vi "Main.vi"() -> ()   [LabVIEW 2018, in "login.lvlib"]
doc: "This template is based from the Queued Message Handler design pattern and the Queued Message Handler Project Template that ships with LabVIEW 2014.\n\nThe main difference is that the Queue is private to this module and communication between modules is done via Broadcast and Request events.\n\nRequest events are wrapped via public API methods and are handled in the Event handler loop in this VI.\nAny module can register for Broadcast events sent by this module.\n\nThe Event Handling Loop generates messages based on user interface actions.\n\nThe Message Handling Loop processes messages generated by the Event Handling Loop, or by other messages. The messages are string values, so new messages can be added easily to the Message Cases case structure in the Message Handling Loop. Each message cluster can also provide an optional value for Message Data, which is a variant that can be converted to whatever message-specific data is required.\n_____\nBased on Delacor QMH Project Template 3.1.0.34."
uses:
  login.lvlib
  <vilib>/Delacor/Delacor QMH/Libraries/Module Admin_class/Delacor_lib_QMH_Module Admin.lvclass
  <vilib>/MGI/Panel Manager/Panel/Panel/Panel.lvclass
  <vilib>/Utility/miscctls.llb/LVPointTypeDef.ctl
  Module Data--cluster.ctl
  Database/Database_access.lvclass
  Path_Management_Class/Path_management.lvclass
  <vilib>/Delacor/Delacor QMH/Libraries/Message Queue_class/Delacor_lib_QMH_Message Queue.lvclass/Delacor_lib_QMH_Message Queue.ctl
  Stop Argument--cluster.ctl
  <vilib>/Delacor/Delacor QMH/Libraries/Module Admin_class/Delacor_lib_QMH_Module Admin.lvclass/Delacor_lib_QMH_Module Admin.ctl
  hid_panl Argument--cluster.ctl
  <vilib>/Utility/miscctls.llb/LVRowAndColumnTypeDef.ctl
  Path_Management_Class/Register_path.ctl
  <vilib>/Delacor/Delacor QMH/Libraries/Message Queue_class/Delacor_lib_QMH_Enqueue Message (Single).vi
  <vilib>/Delacor/Delacor QMH/Libraries/Module Admin_class/Delacor_lib_QMH_Get External Launch.vi
  <vilib>/MGI/Panel Manager/Panel/Panel/Window/Window.lvclass
  C:/Program Files (x86)/National Instruments/LabVIEW 2018/vi.lib/MGI/Panel Manager/Panel/Panel/Panel.lvclass
  <vilib>/Utility/error.llb/Error Cluster From Error Code.vi
  <vilib>/MGI/Panel Manager/Panel/Panel/Window/Window.vi
  <vilib>/ErrorRing/Error Ring.xnode
  <vilib>/Delacor/Delacor QMH/Libraries/Message Queue_class/Delacor_lib_QMH_Message Queue.lvclass
  <vilib>/MGI/Panel Manager/Panel/Panel Helper/Panel Helper.lvclass
  <vilib>/MGI/Panel Manager/Panel/Panel.lvlib
panel:
  in  "Panel 2":refnum<class "Panel.lvclass"> caption="Panel (Window)"
  in  "管理返回":bool
  in  "注册取消":bool
  in  "注册确定":bool
  in  "authority":u16(ring) items=["管理员", "操作员"]
  in  "Password":string
  in  "Name":string
  in  "用户信息":i32[](listbox)
  in  "注册":bool
  in  "删除":bool
  in  "改密确定":bool
  in  "改密取消":bool
  in  "确认新密码":string
  in  "新密码":string
  in  "旧密码":string
  out "用户名 2":string
  in  "返回":bool
  out "用户":string
  in  "退出登录":bool
  in  "用户管理":bool
  in  "修改密码":bool
  in  "登录取消":bool
  in  "登陆确定":bool
  in  "密码":string
  in  "用户名":string(combo)
  in  "Panel":refnum<class "Panel.lvclass">
  in  "Simulate MHL Error":bool
  in  "Simulate EHL Error":bool
  out "error out":errorcluster
  in  "Module Admin":refnum<class "Delacor_lib_QMH_Module Admin.lvclass">
  out "Status":string
  # "XXX登录系统"
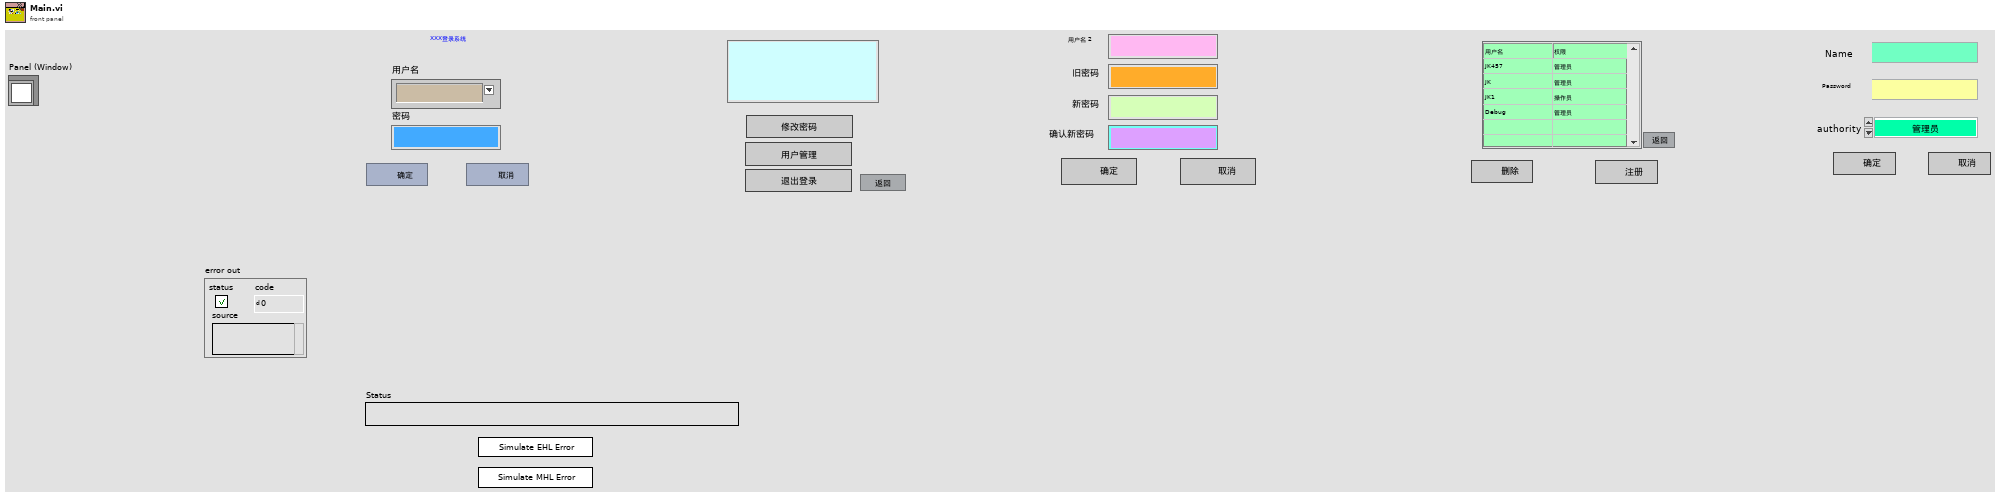
[diagram p1: front panel]
types:
  T1 = typedef "LVPointTypeDef.ctl" = cluster{"Horizontal":i16, "Vertical":i16}
  T2 = typedef "login.lvlib/Request Events--cluster.ctl" = cluster{"Stop Module":refnum<user-event>, "Show Panel":refnum<user-event>, "Hide Panel":refnum<user-event>, "Get Module Execution Status":refnum<user-event>, "Show Diagram":refnum<user-event>, "Change Panel":refnum<user-event>, "原点":refnum<user-event>, "hid_panl":refnum<user-event>}
  T3 = typedef "Panel.lvlib/Panel Helper.lvclass/Panel Events.ctl" = cluster{"My Panel":refnum<user-event>, "Top Level Initialized":refnum<user-event>}
  T4 = typedef "login.lvlib/Broadcast Events--cluster.ctl" = cluster{"Module Did Init":refnum<user-event>, "Status Updated":refnum<user-event>, "Error Reported":refnum<user-event>, "Module Did Stop":refnum<user-event>, "Update Module Execution Status":refnum<user-event>}
  T5 = typedef "login.lvlib/Module Data--cluster.ctl" = cluster{"Status":string, "Database_access.lvclass":refnum<class "Database_access.lvclass">, "Path_management.lvclass":refnum<class "Path_management.lvclass">, "user-passwords":string}
  T6 = typedef "login.lvlib/Stop Argument--cluster.ctl" = cluster{"Origin":string, "Exit via Stop Module Req?":bool, "Wait for Module to stop?":bool}
  T7 = typedef "login.lvlib/原点 Argument--cluster.ctl" = cluster{"x":dbl, "y":dbl}
  T8 = typedef "login.lvlib/hid_panl Argument--cluster.ctl" = cluster{"布尔":bool}
  T9 = typedef "LVRowAndColumnTypeDef.ctl" = cluster{"Row":i32, "Column":i32}
  T10 = typedef "Path_management.lvclass/Register_path.ctl" = string
  T11 = enum32{"invalid lock state", "Not Locked", "Locked (No Password)", "Password-protected"}
  T12 = enum32{"Invalid", "Standard", "Closed", "Hidden", "Minimized", "Maximized"}
  T13 = typedef "login.lvlib/登录蔟.ctl" = cluster{"登录名":string, "权限":string}
  T14 = cluster{"Name":string, "字符串":string, "Password":string}
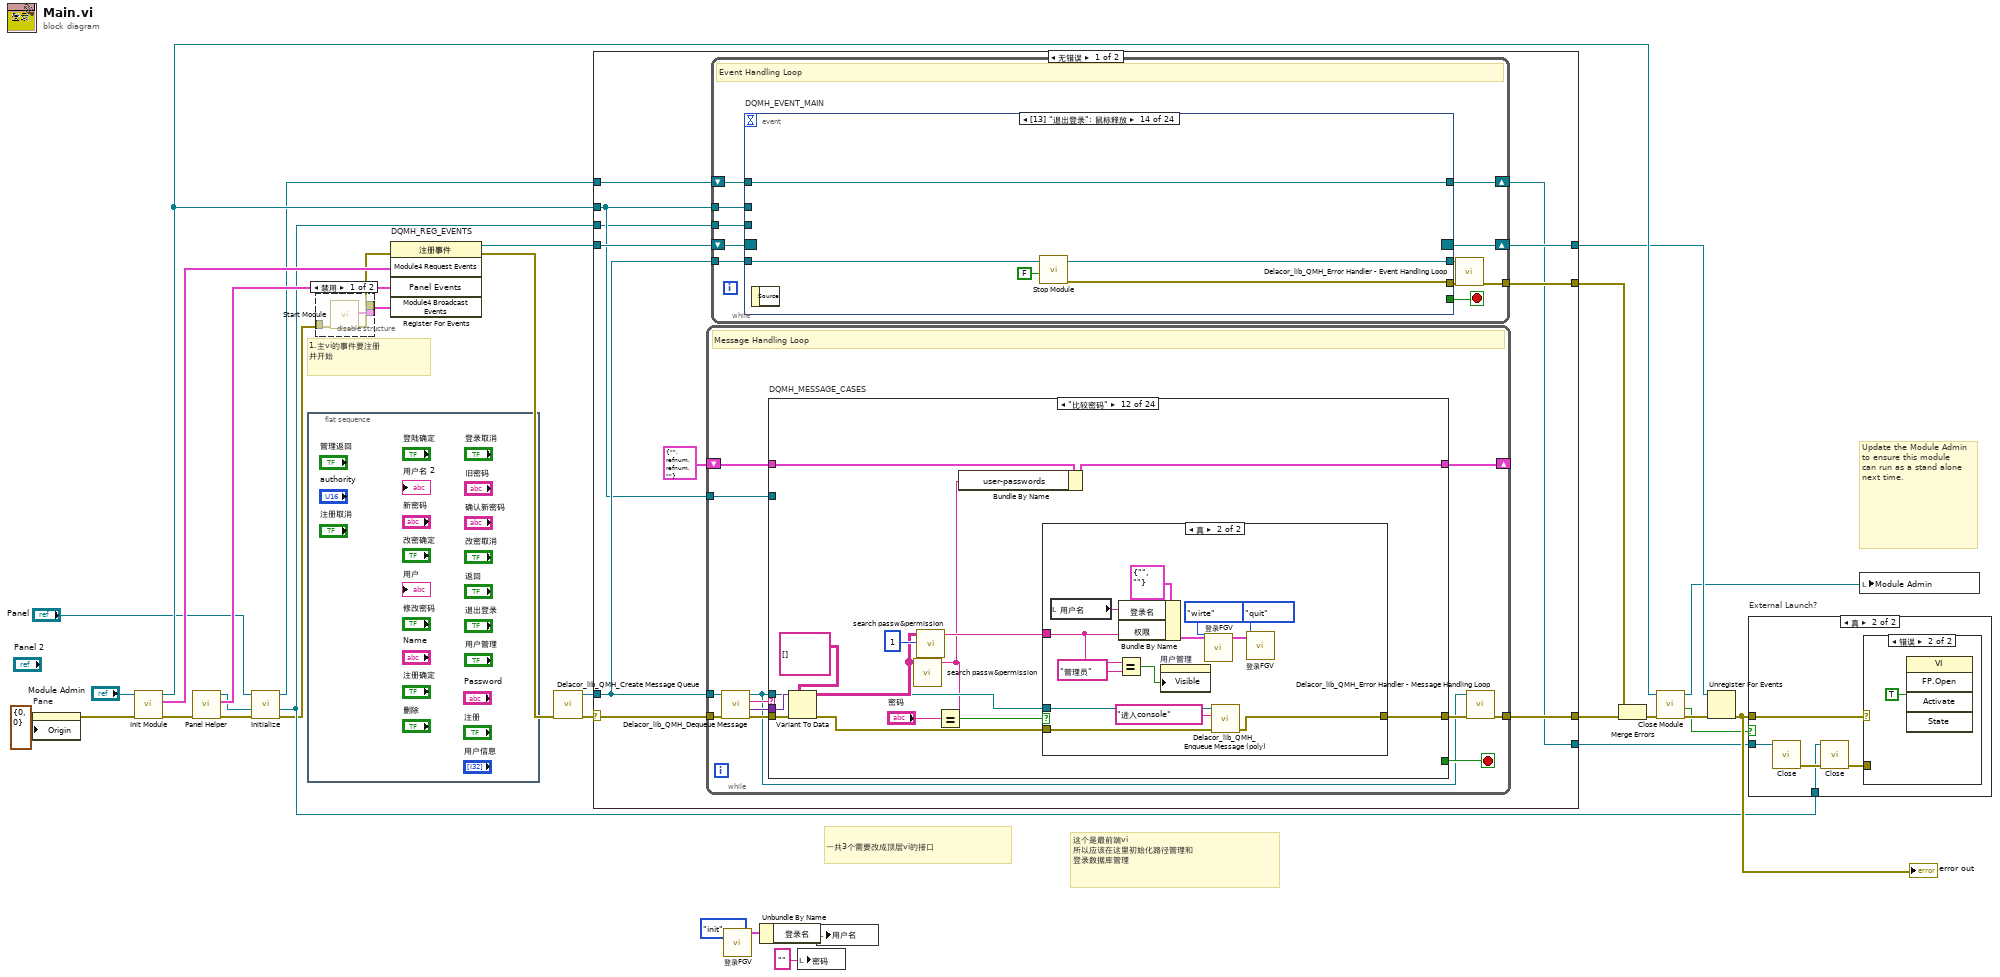
[diagram p0: block diagram]
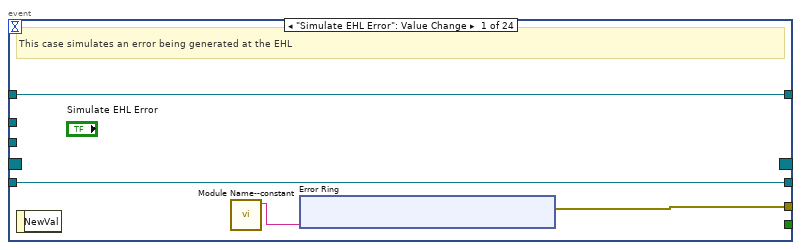
[diagram p5: hidden frame]
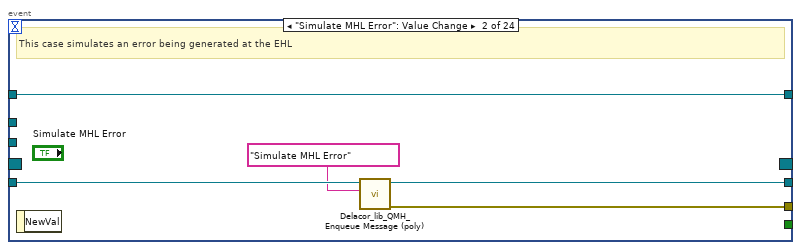
[diagram p6: hidden frame]
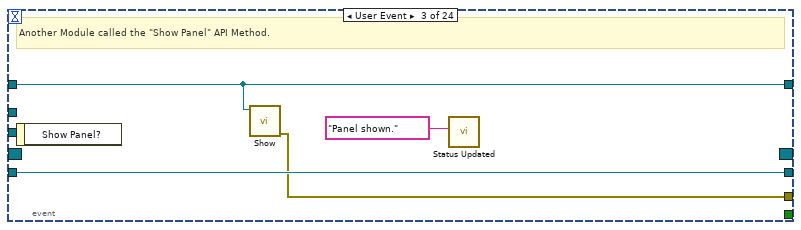
[diagram p7: hidden frame]
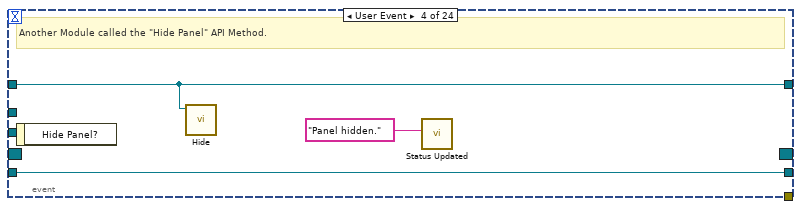
[diagram p8: hidden frame]
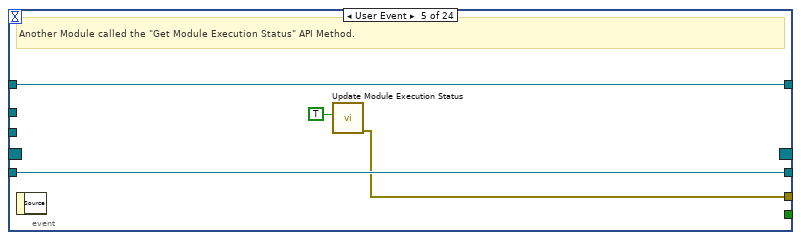
[diagram p9: hidden frame]
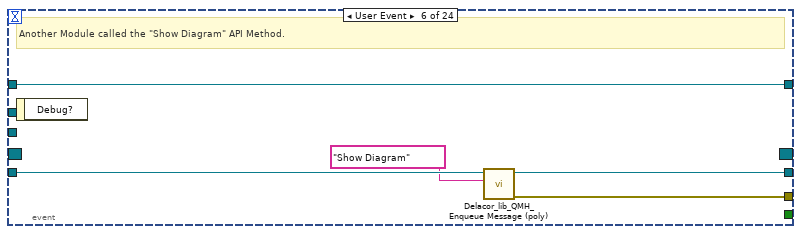
[diagram p10: hidden frame]
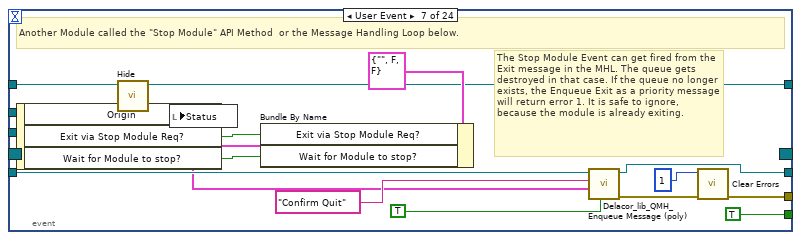
[diagram p11: hidden frame]
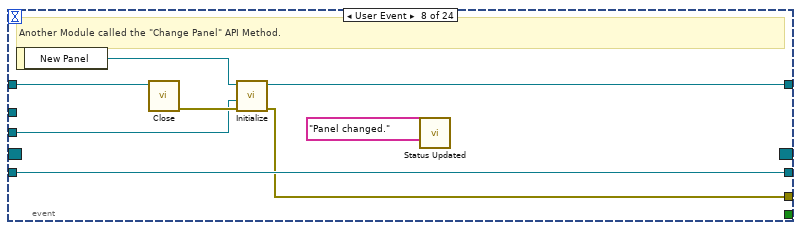
[diagram p12: hidden frame]
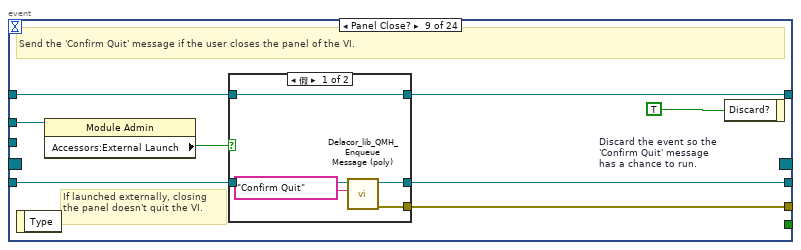
[diagram p13: hidden frame]
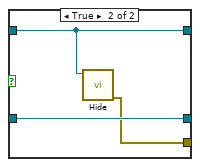
[diagram p14: hidden frame]
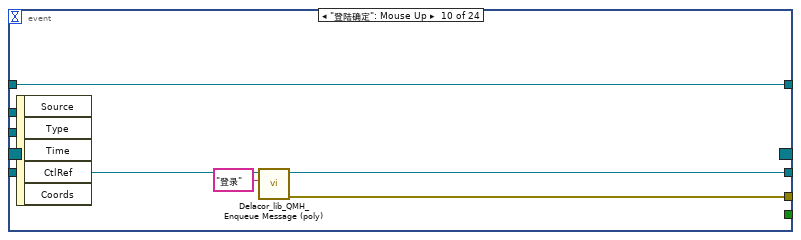
[diagram p15: hidden frame]
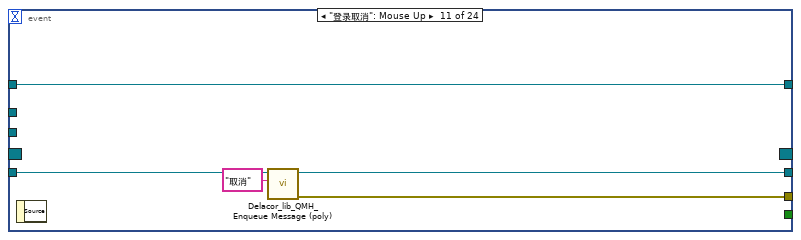
[diagram p16: hidden frame]
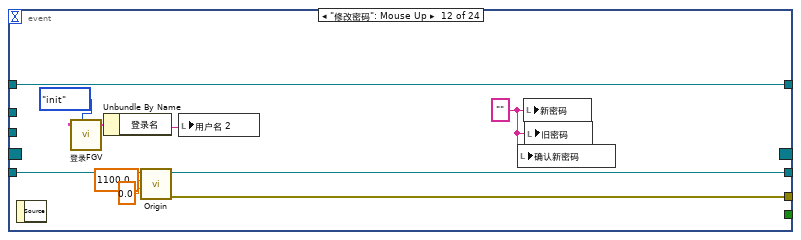
[diagram p17: hidden frame]
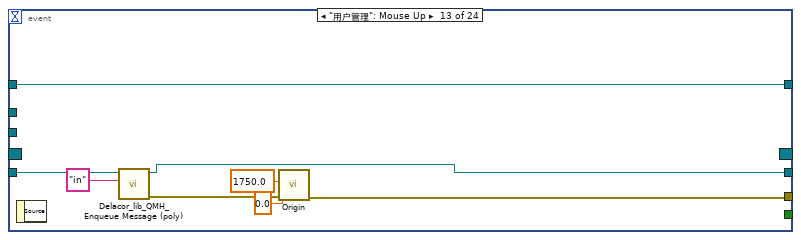
[diagram p18: hidden frame]
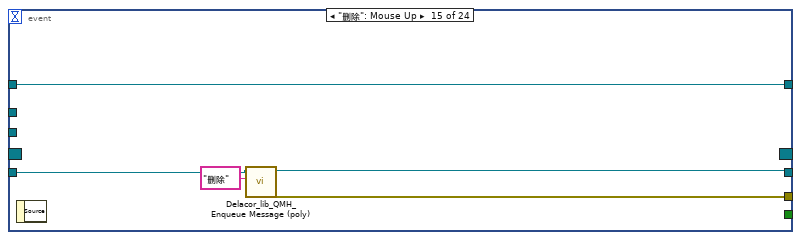
[diagram p19: hidden frame]
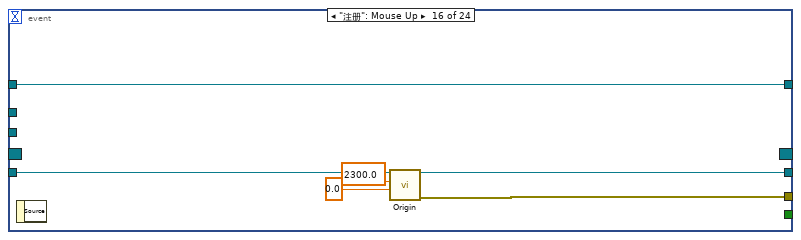
[diagram p20: hidden frame]
diagram:
  # "这个是最前端vi\n所以应该在这里初始化路径管理和\n登录数据库管理"
  # "一共3个需要改成顶层vi的接口"
  # "1.主vi的事件要注册\n并开始"
  # "Update the Module Admin to ensure this module can run as a stand alone next time."
  n1 = property on="Pane" class="Pane"("Origin"=T1 {"Horizontal"=0, "Vertical"=0}) -> (error out=w12:errorcluster)  [unwired: 2 in, 1 out]
  n2 = call "Init Module.vi"("error in (no error)"=w12, "Singleton Module Admin in"="Module Admin") -> ("error out"=w19:errorcluster, "Module4 Request Events"=w28:T2, "Singleton Module Admin out"=w32:refnum<class "Delacor_lib_QMH_Module Admin.lvclass">)  [unwired: 7 in]
  n3 = call <vilib>:"Panel Helper.vi"("Error In"=w19) -> ("Error Out"=w17:errorcluster, "Panel Events"=w18:T3, "Panel Helper out"=w16:refnum<class "Panel Helper.lvclass">)  [unwired: 8 in]
  n4 = call <vilib>:"Initialize.vi"("error in (no error)"=w17, "My Helper in"=w16, "Panel In"="Panel") -> ("error out"=w6:errorcluster, "My Helper out"=w15:refnum<class "Panel Helper.lvclass">, "Panel Out"=w14:refnum<class "Panel.lvclass">)  [unwired: 6 in]
  n5 = flat-sequence {
    frame #0 {
    }
  }
  n6 = disable-structure shown="禁用" {
    disable-tunnel: [w35 _] -> w8
    disable-tunnel: [w34 _] -> w7
    disable-tunnel: w6 -> [w33 _]
    frame Disabled {
      n7 = call "Start Module.vi"("error in (no error)"=w33) -> ("error out"=w34:errorcluster, "Module4 Broadcast Events"=w35:T4)  [unwired: 7 in, 2 out]
    }
    frame Enabled {
    }
  }
  n8 = register-events "DQMH_REG_EVENTS"(error in=w7, w28, w18, w8) -> (reference out=w29:refnum<event-registration>, error out=w5:errorcluster)  [unwired: 1 in]
  n9 = call <vilib>:"Delacor_lib_QMH_Create Message Queue.vi"("error in"=w5) -> ("error out"=w21:errorcluster, "Message Queue"=w27:refnum<class "Delacor_lib_QMH_Message Queue.lvclass">)  [unwired: 9 in]
  n10 = case shown="无错误" w21 {
    selector: w21 -> [w40 w566]
    tunnel: [w46 w566] -> w31
    tunnel: [w45 w571] -> w30
    tunnel: w29 -> [w43 w571]
    tunnel: w27 -> [w42 _]
    tunnel: [w41 _] -> w10
    tunnel: w32 -> [w39 w567]
    tunnel: w14 -> [w37 w563]
    tunnel: w15 -> [w38 _]
    tunnel: [w36 w563] -> w20
    frame No Error {
      n11 = while {
        tunnel: w42 -> [w219]
        shift-right: [w225] -> _
        shift-left: T5 {"Status"="", "Database_access.lvclass"=refnum, "Path_management.lvclass"=refnum, "user-passwords"=""} ("Data Cluster") -> [w226]
        tunnel: w40 -> [w223]
        tunnel: [w217] -> w46
        tunnel: w39 -> [w216]
        stop <- w224 stop-if-true
        # "Message Handling Loop"
        n12 = call-dynamic "Delacor_lib_QMH_Dequeue Message.vi"("error in"=w223, "Message Queue in"=w219) -> ("error out"=w222:errorcluster, "Message Data"=w220:variant, "Message"=w221:string, "Message Queue out"=w218:refnum<class "Delacor_lib_QMH_Message Queue.lvclass">)  [unwired: 6 in]
        n13 = case "DQMH_MESSAGE_CASES" shown="\"比较密码\"" w221 {
          selector: w221 -> [_ _ _ _ _ _ _ _ _ _ _ _ _ _ _ _ _ _ _ _ _ _ _ w552]
          tunnel: w218 -> [w229 w242 w262 _ _ _ _ _ _ _ w351 w373 _ _ w414 _ w463 w471 _ _ w516 w532 w548 _]
          tunnel: w222 -> [w231 w244 w261 w287 w299 w303 w321 w336 w344 w347 w349 w383 w402 w409 w415 w441 w464 w470 w500 w505 w522 w536 w550 _]
          tunnel: [w235 w249 w259 w280 w300 w302 w319 w334 w342 w345 w348 w374 w400 w406 w413 w439 w455 w475 w498 w503 w513 w534 w544 w553] -> w227
          tunnel: w226 -> [w240 w247 w265 w289 w301 w304 w320 w335 w343 w346 w350 w384 w403 w410 w417 w450 w461 w473 w499 w504 w521 w535 w547 w554]
          tunnel: [w239 w246 w264 w289 w301 w304 w320 w335 w343 w346 w350 w372 w403 w410 w417 w450 w461 w473 w499 w504 w521 w535 w547 w554] -> w225
          tunnel: [_ _ _ _ _ _ _ _ _ _ _ _ _ _ _ _ _ _ _ _ _ _ w546 _] -> w224
          tunnel: w220 -> [_ _ _ _ w298 _ _ w333 w341 _ _ w382 _ _ _ _ _ _ _ _ w520 _ w543 _]
          tunnel: w216 -> [w233 _ _ _ _ _ _ _ _ _ _ _ _ _ _ _ _ _ _ _ w515 _ w538 _]
          frame "Initialize" {
            w238 = "Initial Message" ("Initial Message")
            # "#CodeNeeded - Initialize the appearance of the front panel."
            # "#CodeNeeded - Initialize your state data here."
            # "Initialize - Any operation that needs to be done before the module can receive messages. Synchronize Caller Events.vi will inform Start Module.vi that the module has launched and is ready to receive messages. Module Did Init.vi will broadcast that the module initialized."
            n14 = call-poly <vilib>:"Delacor_lib_QMH_Enqueue Message (poly).vi"("error in"=w231, "Message"="init", "Message Queue in"=w229) -> ("error out"=w230:errorcluster)  [unwired: 7 in, 1 out]
            n15 = call "Show Panel.vi"("error in (no error)"=w230) -> ("error out"=w232:errorcluster)  [unwired: 10 in]
            n16 = call "Synchronize Caller Events.vi"("error in (no error)"=w232, "Singleton Module Admin in"=w233) -> ("error out"=w234:errorcluster)  [unwired: 8 in, 1 out]
            n17 = Bundle By Name(cluster=w240, "Status"=w238) -> (w239:T5)
            n18 = local write "Status"(w238) -> ()
            n19 = call "Module Name--constant.vi"() -> ("Module Name"=w236:string)  [unwired: 11 in]
            n20 = call "Module Did Init.vi"("error in (no error)"=w234, "Initialized?"=TRUE, "Origin"=w236) -> ("error out"=w235:errorcluster)  [unwired: 8 in]
          }
          frame "init" {
            n21 = call-poly <vilib>:"Delacor_lib_QMH_Enqueue Message (poly).vi"("error in"=w244, "Message"="ini", "Message Queue in"=w242) -> ("error out"=w243:errorcluster)  [unwired: 7 in, 1 out]
            n22 = in-place {
              in-place-border: w243 -> [w254]
              in-place-border: [w253] -> w245
              # "初始化路径管理类"
              n23 = in-place-cluster #1(w247) -> ("Path_management.lvclass"=w256:refnum<class "Path_management.lvclass">)
              n24 = call-dynamic "INIT_path.vi"("error in (no error)"=w254, "Path_management 输入"=w256) -> ("error out"=w253:errorcluster, "Path_management 输出"=w255:refnum<class "Path_management.lvclass">)  [unwired: 8 in]
              n25 = in-place-cluster #1("Path_management.lvclass"=w255) -> (w246:T5)
            }
            n26 = call-poly <vilib>:"Panel Type Selector.vi"("Default Title"="Window Test") -> ("error out"=w250:errorcluster, "Window out"=w251:refnum<class "Window.lvclass">)  [unwired: 9 in]
            n27 = call "Change Panel.vi"("error in (no error)"=w250, "New Panel"=w251) -> ("error out"=w248:errorcluster)  [unwired: 9 in]
            n28 = Merge Errors(w245, w248, w243) -> (w249:errorcluster)
          }
          frame "ini" {
            n29 = call-poly <vilib>:"Delacor_lib_QMH_Enqueue Message (poly).vi"("error in"=w261, "Message"="in", "Message Queue in"=w262) -> ("error out"=w260:errorcluster)  [unwired: 7 in, 1 out]
            n30 = in-place {
              in-place-border: w260 -> [w275]
              in-place-border: [w274] -> w259
              # "读出所有账户名"
              n31 = in-place-cluster #2(w265) -> ("Database_access.lvclass"=w278:refnum<class "Database_access.lvclass">)
              n32 = call "Take_Path.vi"("组合框"=T10 "登录数据库路径") -> ("Your_Path"=w277:path)  [unwired: 10 in]
              n33 = call-dynamic "INIT-Connect.vi"("error in (no error)"=w275, "database-path"=w277, "Database_access 输入"=w278) -> ("error out"=w274:errorcluster, "Database_access 输出"=w276:refnum<class "Database_access.lvclass">)  [unwired: 7 in]
              n34 = in-place-cluster #2("Database_access.lvclass"=w276) -> (w264:T5)
            }
            n35 = for {
              tunnel: T9 {"Row"=0, "Column"=0} ("活动单元格:活动单元格") -> [w268]
              tunnel: i32[] [0, 1] -> [w267] mode=indexing
              n36 = for {
                N: 99 -> [_]
                tunnel: w268 -> [w271]
                tunnel: w267 -> [w269]
                i -> [w270]
                n37 = Bundle By Name(cluster=w271, "Column"=w269, "Row"=w270) -> (w272:T9)
                n38 = property on="用户信息" class="MCListbox (严格)"("ActiveCell"=w272, "Justify"=enum16{"Left", "Center", "Right"}."Center" ("活动单元格:单元格对齐")) -> ()  [unwired: 2 in, 2 out]
              }
            }
          }
          frame "in" {
            n39 = Unbundle By Name(w289) -> ("Database_access.lvclass"=w288:refnum<class "Database_access.lvclass">)
            n40 = call-dynamic "Read_database.vi"("error in (no error)"=w287, "columns"=string[] ["User_Name", "User_Right"] ("table"), "table"="User_Table", "Database_access 输入"=w288) -> ("error out"=w285:errorcluster, "data"=w286:variant[][])  [unwired: 5 in, 1 out]
            n41 = call "StringArr-type"("error in (no error)"=w285, "database variant"=w286) -> ("error out"=w284:errorcluster, "data"=w283:string[][])  [unwired: 8 in]
            n42 = Index Array(array=w283, index (col)=0 ("禁用的索引 (列)")) -> (element=w293:string[])  [unwired: 1 in]
            n43 = property on="用户信息" class="MCListbox (严格)"("ItemNames"=w283) -> (error out=w281:errorcluster)  [unwired: 2 in, 1 out]
            n44 = property on="用户名" class="CmbBox"(error in=w284, "Strings[]"=w293) -> (error out=w282:errorcluster)  [unwired: 1 in, 1 out]
            n45 = Merge Errors(w282, w281) -> (w280:errorcluster)
          }
          frame "Update Display" {
            # "Broadcast updated status to any VI registered to listen to this module's broadcast events."
            # "Convert the message data to a string to display in the Status indicator."
            # "#CodeRecommended - If you wish to decouple the Message Handling Loop from your user interface, consider creating User Events (like the \"Stop\" event in this VI) to message the Event Handling Loop whenever the user interface needs updating."
            # "Update Display - Update user interface here."
            n46 = Variant To Data(error in=w299, type="" ("空字符串常量"), Variant=w298) -> (data=w296:string, error out=w295:errorcluster)
            "Status" <- w296
            n47 = call "Status Updated.vi"("error in (no error)"=w295, "Status"=w296) -> ("error out"=w294:errorcluster)  [unwired: 9 in]
            n48 = Merge Errors(w294) -> (w300:errorcluster)
          }
          frame "Show Diagram" {
            # "Show Diagram - Show the block diagram of this VI. Used as a debugging tool. There is a button in the module tester that fires the Show Diagram request, which runs this message. Note that the diagram will not be displayed if it is password-protected and the password is not in the cache."
            n49 = disable-structure shown="RUN_TIME_ENGINE==False" {
              disable-tunnel: [w312 w318] -> w302
              disable-tunnel: w303 -> [w311 w318]
              frame condition #0 (active) {
                # "functionality not available in exe"
                n50 = invoke class="VI" method="Lock State.Get"(error in=w311) -> (error out=w310:errorcluster, "Get Lock State"=w309:T11, "pwd in cache"=w306:bool)  [unwired: 3 in, 1 out]
                n51 = Equal?(x=T11."Password-protected", y=w309) -> (x = y?=w307:bool)
                n52 = Compound Arithmetic op=AND(w307, invert w306) -> (w305:bool)
                n53 = case shown="假" w305 {
                  tunnel: [w315 w317] -> w312
                  tunnel: w310 -> [w313 w317]
                  frame False {
                    n54 = property class="VI"(error in=w313, "BDWin.Open"=TRUE ("Block Diagram Window:Open")) -> (error out=w315:errorcluster)  [unwired: 1 in, 1 out]
                    n55 = call "Status Updated.vi"("Status"="Block Diagram shown." ("format string")) -> ()  [unwired: 10 in, 1 out]
                  }
                  frame True {
                    # "Password-protected VI, and the password is not in the cache. Do not show the diagram."
                  }
                }
              }
              frame condition #1 {
              }
            }
          }
          frame "--- Module Specific ---" {
            # "Separator -- The following cases handle messages specific to this Module."
            n56 = Merge Errors(w321) -> (w319:errorcluster)
          }
          frame "原点" {
            # "原点滚动"
            n57 = Variant To Data(error in=w336, type=T7 {"x"=0.0, "y"=0.0} ("原点 Argument"), Variant=w333) -> (data=w331:T7, error out=w334:errorcluster)
            n58 = Unbundle By Name(w331) -> ("x"=w328:dbl, "y"=w327:dbl)
            n59 = Bundle By Name(cluster=T1 {"Horizontal"=0, "Vertical"=0} ("原点"), "Horizontal"=w328, "Vertical"=w327) -> (w329:T1)
            n60 = call "登录FGV.vi"("枚举"=enum16{"init", "quit", "read", "wirte"}."read") -> ("wirte 2"=w325:T13)  [unwired: 10 in]
            n61 = Unbundle By Name(w325) -> ("登录名"=w324:string)
            n62 = property on="Pane" class="Pane"("Origin"=w329) -> ()  [unwired: 2 in, 2 out]
            n63 = Format Into String(format string="欢迎--QAQ--\n%s\n花花Cillao花花" ("格式字符串"), w324) -> (resulting string=w323:string)  [unwired: 2 in, 1 out]
            n64 = local write "用户"(w323) -> ()
          }
          frame "hid_panl" {
            # "内部调用前面板关闭会出问题，我就自己写了一个简单的\n这个只内部调用"
            n65 = Variant To Data(error in=w344, type=T8 {"布尔"=FALSE} ("hid_panl Argument"), Variant=w341) -> (data=w339:T8, error out=w342:errorcluster)
            n66 = Unbundle By Name(w339) -> ()  [unwired: 1 out]
            n67 = control-ref of="本VI"() -> (w338:refnum<vi>)
            n68 = invoke class="VI" method="FP.Open"(reference=w338, "State"=T12."Hidden" ("状态")) -> ()  [unwired: 3 in, 5 out]
          }
          frame "---Copy This Frame---" {
            # "Duplicate this frame when creating new messages.  Change this comment in the duplicated frame to describe this message."
            n69 = Merge Errors(w347) -> (w345:errorcluster)
          }
          frame "登录" {
            n70 = Empty String/Path?(string/path="用户名") -> (empty?=w353:bool)
            n71 = case shown="假" w353 {
              tunnel: "用户名" -> [w362 _]
              tunnel: w351 -> [w368 _]
              tunnel: w350 -> [w367 _]
              tunnel: w349 -> [w360 w369]
              tunnel: [w358 w369] -> w348
              frame False {
                n72 = Unbundle By Name(w367) -> ("Database_access.lvclass"=w366:refnum<class "Database_access.lvclass">)
                n73 = Format Into String(format string=" where User_Name ='%s'" ("condition"), error in=w360, w362) -> (resulting string=w361:string, error out=w359:errorcluster)  [unwired: 1 in]
                n74 = call-dynamic "Read_database.vi"("condition"=w361, "error in (no error)"=w359, "table"="User_Table", "Database_access 输入"=w366) -> ("error out"=w356:errorcluster, "data"=w357:variant[][])  [unwired: 5 in, 1 out]
                n75 = call "StringArr-type"("error in (no error)"=w356, "database variant"=w357) -> ("error out"=w355:errorcluster, "data"=w354:string[][])  [unwired: 8 in]
                n76 = call-poly <vilib>:"Delacor_lib_QMH_Enqueue Message (poly).vi"("error in"=w355, "Message Data"=w354, "Message"="比较密码", "Message Queue in"=w368) -> ("error out"=w358:errorcluster)  [unwired: 6 in, 1 out]
              }
              frame True {
                n77 = One Button Dialog(message="我都弄成让你选的了\n你还不输入的话很难办啊盆友" ("消息")) -> ()  [unwired: 1 in, 1 out]
              }
            }
          }
          frame "比较密码" {
            n78 = Variant To Data(error in=w383, type=string[][] [] ("table"), Variant=w382) -> (data=w378:string[][], error out=w375:errorcluster)
            n79 = call "search passw&permission.vi"("数组"=w378) -> ("元素"=w371:string)  [unwired: 9 in, 1 out]
            n80 = call "search passw&permission.vi"("索引"=1, "数组"=w378) -> ("元素"=w376:string)  [unwired: 8 in, 1 out]
            n81 = Equal?(x=w371, y="密码") -> (x = y?=w377:bool)
            n82 = Bundle By Name(cluster=w384, "user-passwords"=w371) -> (w372:T5)
            n83 = case shown="真" w377 {
              tunnel: w376 -> [_ w389]
              tunnel: w375 -> [w386 w393]
              tunnel: [w386 w392] -> w374
              tunnel: w373 -> [_ w391]
              frame False {
                n84 = One Button Dialog(message="是本人吗就乱登录" ("消息")) -> ()  [unwired: 1 in, 1 out]
              }
              frame True {
                n85 = local read "用户名"() -> (w394:string)
                n86 = Equal?(x=w389, y="管理员") -> (x = y?=w388:bool)
                n87 = Bundle By Name(cluster=T13 {"登录名"="", "权限"=""} ("wirte"), "登录名"=w394, "权限"=w389) -> (w398:T13)
                n88 = property on="用户管理" class="Bool (严格)"("Visible"=w388) -> ()  [unwired: 2 in, 2 out]
                n89 = call "登录FGV.vi"("枚举"=enum16{"init", "quit", "read", "wirte"}."wirte", "wirte"=w398) -> ("wirte 2"=w399:T13)  [unwired: 9 in]
                n90 = call-poly <vilib>:"Delacor_lib_QMH_Enqueue Message (poly).vi"("error in"=w393, "Message"="进入console", "Message Queue in"=w391) -> ("error out"=w392:errorcluster)  [unwired: 7 in, 1 out]
                n91 = call "登录FGV.vi"("枚举"=enum16{"init", "quit", "read", "wirte"}."quit", "wirte"=w399) -> ()  [unwired: 9 in, 1 out]
              }
            }
          }
          frame "进入console" {
            # "2.进入时候打开主vi面板"
            # "隐藏自己"
            # "展示main"
            n92 = call "Hide Panel.vi"("error in (no error)"=w402) -> ("error out"=w401:errorcluster)  [unwired: 10 in]
            n93 = disable-structure shown="禁用" {
              disable-tunnel: w401 -> [w405 _]
              disable-tunnel: [w404 _] -> w400
              frame Disabled {
                n94 = call "Show Panel.vi"("error in (no error)"=w405) -> ("error out"=w404:errorcluster)  [unwired: 10 in]
              }
              frame Enabled {
              }
            }
          }
          frame "取消" {
            # "3.停止主VI"
            # "停止"
            # "隐藏自己"
            # "为什么要先隐藏\n因为再DQMH中只有点X号才能\n出发关闭前面板，否则会变成停止，"
            n95 = call "Hide Panel.vi"("error in (no error)"=w409) -> ("error out"=w408:errorcluster)  [unwired: 10 in]
            n96 = disable-structure shown="禁用" {
              disable-tunnel: w408 -> [w412 _]
              disable-tunnel: [w411 _] -> w407
              frame Disabled {
                n97 = call "Stop Module.vi"("error in (no error)"=w412) -> ("error out"=w411:errorcluster)  [unwired: 10 in]
              }
              frame Enabled {
              }
            }
            n98 = call "Stop Module.vi"("error in (no error)"=w407) -> ("error out"=w406:errorcluster)  [unwired: 10 in]
          }
          frame "修改密码" {
            w423 = "" ("y")
            n99 = local read "确认新密码"() -> (w424:string)
            n100 = Unbundle By Name(w417) -> ("user-passwords"=w416:string)
            n101 = local read "新密码"() -> (w418:string)
            n102 = Equal?(x=w418, y=w424) -> (x = y?=w422:bool)
            n103 = Not Equal?(x=w418, y=w423) -> (x != y?=w421:bool)
            n104 = Not Equal?(x=w423, y=w424) -> (x != y?=w420:bool)
            n105 = local read "旧密码"() -> (w426:string)
            n106 = Compound Arithmetic op=AND ("复合运算")(w422, w421, w420) -> (w419:bool)
            n107 = Equal?(x=w416, y=w426) -> (x = y?=w425:bool)
            n108 = case shown="真" w425 {
              tunnel: w419 -> [_ w432]
              tunnel: w418 -> [_ _]
              tunnel: w415 -> [w427 w430]
              tunnel: w414 -> [_ w431]
              tunnel: [w427 w429] -> w413
              frame False {
                n109 = One Button Dialog(message="要输入正确原始密码\n才可以呦" ("消息")) -> ()  [unwired: 1 in, 1 out]
              }
              frame True {
                n110 = case shown="真" w432 {
                  tunnel: w431 -> [_ w438]
                  tunnel: w430 -> [w433 w437]
                  tunnel: [w433 w435] -> w429
                  frame False {
                    n111 = One Button Dialog(message="两次输的\n不一样啊" ("消息")) -> ()  [unwired: 1 in, 1 out]
                  }
                  frame True {
                    n112 = call-poly <vilib>:"Delacor_lib_QMH_Enqueue Message (poly).vi"("error in"=w437, "Message"="修改数据库", "Message Queue in"=w438) -> ("error out"=w435:errorcluster)  [unwired: 7 in, 1 out]
                  }
                }
              }
            }
          }
          frame "修改数据库" {
            n113 = Unbundle By Name(w450) -> ("Database_access.lvclass"=w449:refnum<class "Database_access.lvclass">)
            n114 = local read "用户名 2"() -> (w444:string)
            n115 = Format Into String(format string="Where User_Name='%S'", error in=w441, w444) -> (resulting string=w443:string, error out=w442:errorcluster)  [unwired: 1 in]
            n116 = local read "新密码"() -> (w446:string)
            n117 = call-dynamic "Update_database.vi"("data"=w446, "condition"=w443, "error in (no error)"=w442, "columns"=string[] ["User_Password"], "table"="User_Table", "Database_access 输入"=w449) -> ("error out"=w440:errorcluster)  [unwired: 4 in, 1 out]
            n118 = call "Origin.vi"("error in"=w440, "数值 2"=0.0, "数值"=550.0) -> ("error out"=w439:errorcluster)  [unwired: 8 in]
            n119 = One Button Dialog(message="密码已修改" ("消息"), button name ("OK")="朕知道了" ("按钮名称（“确定”）")) -> ()  [unwired: 1 out]
          }
          frame "删除" {
            n120 = Unbundle By Name(w461) -> ("Database_access.lvclass"=w460:refnum<class "Database_access.lvclass">)
            n121 = call-poly <vilib>:"Delacor_lib_QMH_Enqueue Message (poly).vi"("error in"=w464, "Message"="in", "Message Queue in"=w463) -> ("error out"=w458:errorcluster)  [unwired: 7 in, 1 out]
            n122 = property on="用户信息" class="MCListbox (严格)"() -> ("ItemNames"=w466:string[][], "FocusRow"=w467:i32)  [unwired: 2 in, 2 out]
            n123 = Index Array(array=w466, index (row)=w467) -> (element=w465:string[])  [unwired: 1 in]
            n124 = Index Array(array=w465) -> (element=w456:string)  [unwired: 1 in]
            n125 = call-dynamic "Delete_database.vi"("name"=w456, "error in (no error)"=w458, "Item-name"="User_Name" ("table"), "table"="User_Table", "Database_access 输入"=w460) -> ("error out"=w455:errorcluster)  [unwired: 5 in, 1 out]
          }
          frame "注册确定" {
            n126 = local read "Password"() -> (w468:string)
            n127 = local read "Name"() -> (w474:string)
            n128 = local read "authority"() -> (w477:u16)
            n129 = Empty String/Path?(string/path=w474) -> (empty?=w479:bool)
            n130 = Empty String/Path?(string/path=w468) -> (empty?=w480:bool)
            n131 = call "emur-char.vi"("authority 2"=w477) -> ("字符串"=w476:string)  [unwired: 10 in]
            n132 = Not And(1:w480, 2:w479) -> (0:w478:bool)
            n133 = case shown="真" w478 {
              tunnel: w476 -> [_ w482]
              tunnel: w474 -> [_ w496]
              tunnel: w468 -> [_ w483]
              tunnel: w473 -> [_ w497]
              tunnel: [_ w488] -> w472
              tunnel: w471 -> [_ w487]
              tunnel: w470 -> [_ w495]
              tunnel: [_ w485] -> w469
              frame False {
                n134 = One Button Dialog(message="不能有空的啊" ("消息")) -> ()  [unwired: 1 in, 1 out]
              }
              frame True {
                n135 = Unbundle By Name(w497) -> ("Database_access.lvclass"=w492:refnum<class "Database_access.lvclass">)
                n136 = Bundle("Name"=w496, "字符串"=w482, "Password"=w483) -> (w489:T14)  [unwired: 1 in]
                n137 = call "Origin.vi"("error in"=w495, "数值 2"=0.0, "数值"=1750.0) -> ("error out"=w486:errorcluster)  [unwired: 8 in]
                n138 = call-dynamic "Insert_database.vi"("data"=w489, "columns"=string[] ["User_name", "User_Right", "User_password"], "table"="User_Table", "Database_access 输入"=w492) -> ("error out"=w488:errorcluster)  [unwired: 6 in, 1 out]
                n139 = call-poly <vilib>:"Delacor_lib_QMH_Enqueue Message (poly).vi"("error in"=w486, "Message"="in", "Message Queue in"=w487) -> ("error out"=w485:errorcluster)  [unwired: 7 in, 1 out]
              }
            }
            n140 = Merge Errors(w472, w469) -> (w475:errorcluster)
          }
          frame "--- Exit and Error Handling---" {
            # "Separator - The following cases handle errors and exit messages."
            n141 = Merge Errors(w500) -> (w498:errorcluster)
          }
          frame "Simulate MHL Error" {
            # "Simulate an error occurring at the MHL"
            n142 = call "Module Name--constant.vi"() -> ("Module Name"=w502:string)  [unwired: 11 in]
            n143 = xnode "Error Ring"("参数 0"=w502) -> ("错误输出"=w501:errorcluster)
            n144 = Merge Errors(w505, w501) -> (w503:errorcluster)
          }
          frame "Error" {
            # "#CodeRecommended - If you ever change the name of this \"Error\" message, you'll need to update the name in the Check Loop Error.vi as well."
            # "#CodeRecommended - If the module is running in standalone mode (External Launch = FALSE), this code will pop up an error dialog and call the 'Exit' message if an error occurs. Add more fine-grained error handling here."
            # "Error - Check the error message data and respond accordingly. This message is sent by the \"Error Handler\" VIs at the end of each loop in this application."
            n145 = property class="Module Admin"(reference=w515) -> ("Accessors:External Launch"=w514:bool)  [unwired: 1 in, 2 out]
            n146 = Variant To Data(error in=w522, type=errorcluster {"status"=FALSE, "code"=0, "source"=""} ("error constant"), Variant=w520) -> (data=w523:errorcluster, error out=w518:errorcluster)
            n147 = call "Error Reported.vi"("Error"=w523) -> ()  [unwired: 10 in, 1 out]
            n148 = case shown="假" w514 {
              tunnel: [w528 _] -> w517
              tunnel: w516 -> [w527 _]
              tunnel: w523 -> [w524 _]
              frame False {
                # "If the module is running standalone, then pop up an error dialog and call the \"Exit\" message."
                n149 = call <vilib>:"Simple Error Handler.vi"("error in (no error)"=w524) -> ()  [unwired: 4 in, 5 out]
                n150 = call-poly <vilib>:"Delacor_lib_QMH_Enqueue Message (poly).vi"("Priority Message? (F)"=TRUE, "Message"="Exit", "Message Queue in"=w527) -> ("error out"=w528:errorcluster)  [unwired: 7 in, 1 out]
              }
              frame True {
                # "If the module was launched externally, calling the Error Reported broadcast VI is the only action performed by the \"Error\" message. The module's caller can then process the error appropriately."
              }
            }
            n151 = Merge Errors(w518, w517) -> (w513:errorcluster)
            n152 = local write "error out"(w513) -> ()
          }
          frame "Confirm Quit" {
            # "main停止"
            # "Confirm Quit - Message that can confirm whether or not the user wants to exit the application."
            n153 = call-poly <vilib>:"Delacor_lib_QMH_Enqueue Message (poly).vi"("Priority Message? (F)"=TRUE, "error in"=w536, "Message"="Exit", "Message Queue in"=w532) -> ("error out"=w533:errorcluster)  [unwired: 6 in, 1 out]
            n154 = call "Stop Module.vi"() -> ("error out"=w529:errorcluster)  [unwired: 11 in]
            n155 = Merge Errors(w529, w533) -> (w534:errorcluster)
          }
          frame "Exit" {
            w541 = 91  # 91: not all Exit messages will have an argument
            w546 = TRUE  # Stop the VI
            # "Release the message queue reference"
            # "#CodeNeeded - Add any required cleanup code here"
            # "Exit - Exit the application."
            n156 = Variant To Data(error in=w550, type=T6 {"Origin"="", "Exit via Stop Module Req?"=FALSE, "Wait for Module to stop?"=FALSE} ("Stop Argument"), Variant=w543) -> (data=w539:T6, error out=w542:errorcluster)
            n157 = call <vilib>:"Clear Errors.vi"("error in (no error)"=w542, "specific error code to clear (0: all)"=w541) -> ("error out"=w549:errorcluster)  [unwired: 4 in, 1 out]
            n158 = call-dynamic "Delacor_lib_QMH_Release Message Queue.vi"("error in"=w549, "Message Queue"=w548) -> ("error out"=w545:errorcluster)  [unwired: 9 in]
            n159 = call "Handle Exit.vi"("Stop Argument"=w539, "Admin in"=w538) -> ("error out"=w537:errorcluster)  [unwired: 8 in, 1 out]
            n160 = Merge Errors(w537, w545) -> (w544:errorcluster)
          }
          frame Default {
            # "'Default' case only runs if there is a message that isn't defined in any of the other cases.  Output a programming error."
            n161 = call "Module Name--constant.vi"() -> ("Module Name"=w551:string)  [unwired: 11 in]
            n162 = xnode "Error Ring"("参数 0"=w552, "参数 1"=w551) -> ("错误输出"=w553:errorcluster)
          }
        }
        n163 = call-dynamic "Delacor_lib_QMH_Error Handler - Message Handling Loop.vi"("error in"=w227, "Message Queue in"=w218) -> ("dup error in"=w217:errorcluster)  [unwired: 8 in, 1 out]
      }
      n164 = while {
        tunnel: w42 -> [w57]
        shift-right: [w55] -> w45
        shift-left: w43 -> [w56]
        tunnel: [w51] -> w41
        tunnel: w39 -> [w50]
        tunnel: w38 -> [w49]
        shift-right: [w47] -> w36
        shift-left: w37 -> [w48]
        stop <- w53 stop-if-true
        # "Event Handling Loop"
        n165 = event "DQMH_EVENT_MAIN" shown="[13] \"退出登录\": 鼠标释放" {
          selector: w56 -> [_ _ _ _ _ _ _ _ _ _ _ _ _ _ _ _ _ _ _ _ _ _ _ _]
          dyn-events: [_ _ _ _ _ _ _ _ _ _ _ _ _ _ _ _ _ _ _ _ _ _ _ _] -> w55
          timeout: _ -> [_ _ _ _ _ _ _ _ _ _ _ _ _ _ _ _ _ _ _ _ _ _ _ _]
          tunnel: [_ _ _ _ _ _ TRUE ("Discard?") _ _ _ _ _ _ _ _ _ _ _ _ _ _ _ _ _] -> w53
          tunnel: w57 -> [w61 w73 w77 w80 w84 w89 w101 w111 w118 w131 w136 w142 w150 w158 w162 w168 w173 w177 w183 w187 w192 w196 w207 w215]
          tunnel: [w60 w70 w75 _ w83 w86 w95 w107 w117 w128 w133 w143 w153 w156 w160 w164 w171 w175 w181 w185 w191 w195 w199 w208] -> w54
          tunnel: [w61 w72 w77 w80 w84 w88 w100 w111 w116 w130 w135 w142 w149 w158 w161 w168 w173 w176 w183 w186 w192 w197 w205 w213] -> w52
          tunnel: w50 -> [_ _ _ _ _ _ _ _ w115 _ _ _ _ _ _ _ _ _ _ _ _ _ _ _]
          tunnel: w49 -> [_ _ _ _ _ _ _ w106 _ _ _ _ _ _ _ _ _ _ _ _ _ _ _ _]
          tunnel: w48 -> [w58 w69 w76 w79 w81 w85 w91 w110 w114 w132 w137 w146 w154 w157 w163 w167 w172 w178 w182 w188 w193 w198 w206 w214]
          tunnel: [w58 w69 w76 w79 w81 w85 w91 w105 w113 w132 w137 w146 w154 w157 w163 w167 w172 w178 w182 w188 w193 w198 w206 w214] -> w47
          event "Simulate EHL Error": Value Change {
            # "This case simulates an error being generated at the EHL"
            n166 = event-data() -> ()  [unwired: 1 in, 1 out]
            n167 = call "Module Name--constant.vi"() -> ("Module Name"=w59:string)  [unwired: 11 in]
            n168 = xnode "Error Ring"("参数 0"=w59) -> ("错误输出"=w60:errorcluster)
          }
          event "Simulate MHL Error": Value Change {
            # "This case simulates an error being generated at the EHL"
            n169 = event-data() -> ()  [unwired: 1 in, 1 out]
            n170 = call-poly <vilib>:"Delacor_lib_QMH_Enqueue Message (poly).vi"("Message"="Simulate MHL Error", "Message Queue in"=w73) -> ("error out"=w70:errorcluster, "Message Queue out"=w72:refnum<class "Delacor_lib_QMH_Message Queue.lvclass">)  [unwired: 8 in]
          }
          event User Event {
            # "Another Module called the \"Show Panel\" API Method."
            n171 = event-data() -> ()  [unwired: 1 in, 1 out]
            n172 = call <vilib>:"Show.vi"("Panel in"=w76) -> ("Error Out"=w75:errorcluster)  [unwired: 10 in]
            n173 = call "Status Updated.vi"("Status"="Panel shown." ("format string")) -> ()  [unwired: 10 in, 1 out]
          }
          event User Event {
            # "Another Module called the \"Hide Panel\" API Method."
            n174 = event-data() -> ()  [unwired: 1 in, 1 out]
            n175 = call <vilib>:"Hide.vi"("Panel In"=w79) -> ()  [unwired: 10 in, 1 out]
            n176 = call "Status Updated.vi"("Status"="Panel hidden." ("format string")) -> ()  [unwired: 10 in, 1 out]
          }
          event User Event {
            # "Another Module called the \"Get Module Execution Status\" API Method."
            n177 = event-data() -> ()  [unwired: 1 in, 1 out]
            n178 = call "Update Module Execution Status.vi"("Running?"=TRUE) -> ("error out"=w83:errorcluster)  [unwired: 10 in]
          }
          event User Event {
            # "Another Module called the \"Show Diagram\" API Method."
            n179 = event-data() -> ()  [unwired: 1 in, 1 out]
            n180 = call-poly <vilib>:"Delacor_lib_QMH_Enqueue Message (poly).vi"("Message"="Show Diagram", "Message Queue in"=w89) -> ("error out"=w86:errorcluster, "Message Queue out"=w88:refnum<class "Delacor_lib_QMH_Message Queue.lvclass">)  [unwired: 8 in]
          }
          event User Event {
            # "The Stop Module Event can get fired from the Exit message in the MHL. The queue gets destroyed in that case. If the queue no longer exists, the Enqueue Exit as a priority message will return error 1. It is safe to ignore, because the module is already exiting."
            # "Another Module called the \"Stop Module\" API Method  or the Message Handling Loop below."
            n181 = event-data() -> ("Origin"=w99:string, "Exit via Stop Module Req?"=w93:bool, "Wait for Module to stop?"=w90:bool)  [unwired: 1 in]
            n182 = call <vilib>:"Hide.vi"("Panel In"=w91) -> ()  [unwired: 10 in, 1 out]
            n183 = local write "Status"(w99) -> ()
            n184 = Bundle By Name(cluster=T6 {"Origin"="", "Exit via Stop Module Req?"=FALSE, "Wait for Module to stop?"=FALSE} ("Stop Argument"), "Exit via Stop Module Req?"=w93, "Wait for Module to stop?"=w90) -> (w92:T6)
            n185 = call-poly <vilib>:"Delacor_lib_QMH_Enqueue Message (poly).vi"("Priority Message? (F)"=TRUE, "Message Data"=w92, "Message"="Confirm Quit", "Message Queue in"=w101) -> ("error out"=w96:errorcluster, "Message Queue out"=w100:refnum<class "Delacor_lib_QMH_Message Queue.lvclass">)  [unwired: 6 in]
            n186 = call <vilib>:"Clear Errors.vi"("error in (no error)"=w96, "specific error code to clear (0: all)"=1) -> ("error out"=w95:errorcluster)  [unwired: 4 in, 1 out]
          }
          event User Event {
            # "Another Module called the \"Change Panel\" API Method."
            n187 = event-data() -> ("New Panel"=w109:refnum<class "Panel.lvclass">)  [unwired: 1 in]
            n188 = call-dynamic <vilib>:"Close.vi"("Panel In"=w110) -> ("Error Out"=w108:errorcluster)  [unwired: 10 in]
            n189 = call <vilib>:"Initialize.vi"("error in (no error)"=w108, "My Helper in"=w106, "Panel In"=w109) -> ("error out"=w107:errorcluster, "Panel Out"=w105:refnum<class "Panel.lvclass">)  [unwired: 6 in, 1 out]
            n190 = call "Status Updated.vi"("Status"="Panel changed.") -> ()  [unwired: 10 in, 1 out]
          }
          event Panel Close? {
            w119 = TRUE  # Discard the event so the 'Confirm Quit' message has a chance to run.
            # "If launched externally, closing the panel doesn't quit the VI."
            # "Send the 'Confirm Quit' message if the user closes the panel of the VI."
            n191 = event-data() -> ()  [unwired: 1 in, 1 out]
            n192 = property class="Module Admin"(reference=w115) -> ("Accessors:External Launch"=w112:bool)  [unwired: 1 in, 2 out]
            n193 = case "条件结构" shown="假" w112 {
              tunnel: w118 -> [w124 w127]
              tunnel: [w123 w125] -> w117
              tunnel: [w122 w127] -> w116
              tunnel: w114 -> [w120 w126]
              tunnel: [w120 w126] -> w113
              frame False {
                n194 = call-poly <vilib>:"Delacor_lib_QMH_Enqueue Message (poly).vi"("Message"="Confirm Quit", "Message Queue in"=w124) -> ("error out"=w123:errorcluster, "Message Queue out"=w122:refnum<class "Delacor_lib_QMH_Message Queue.lvclass">)  [unwired: 8 in]
              }
              frame True {
                n195 = call <vilib>:"Hide.vi"("Panel In"=w126) -> ("Error Out"=w125:errorcluster)  [unwired: 10 in]
              }
            }
            n196 = event-data("Discard?"=w119) -> ()  [unwired: 1 in, 1 out]
          }
          event "登陆确定": Mouse Up {
            n197 = event-data() -> ()  [unwired: 1 in, 5 out]
            n198 = call-poly <vilib>:"Delacor_lib_QMH_Enqueue Message (poly).vi"("Message"="登录", "Message Queue in"=w131) -> ("error out"=w128:errorcluster, "Message Queue out"=w130:refnum<class "Delacor_lib_QMH_Message Queue.lvclass">)  [unwired: 8 in]
          }
          event "登录取消": Mouse Up {
            n199 = event-data() -> ()  [unwired: 1 in, 1 out]
            n200 = call-poly <vilib>:"Delacor_lib_QMH_Enqueue Message (poly).vi"("Message"="取消", "Message Queue in"=w136) -> ("error out"=w133:errorcluster, "Message Queue out"=w135:refnum<class "Delacor_lib_QMH_Message Queue.lvclass">)  [unwired: 8 in]
          }
          event "修改密码": Mouse Up {
            w138 = "" ("新密码")
            n201 = event-data() -> ()  [unwired: 1 in, 1 out]
            n202 = call "登录FGV.vi"("枚举"=enum16{"init", "quit", "read", "wirte"}."init") -> ("wirte 2"=w140:T13)  [unwired: 10 in]
            n203 = Unbundle By Name(w140) -> ("登录名"=w139:string)
            n204 = call "Origin.vi"("数值 2"=0.0, "数值"=1100.0) -> ("error out"=w143:errorcluster)  [unwired: 9 in]
            n205 = local write "用户名 2"(w139) -> ()
            n206 = local write "确认新密码"(w138) -> ()
            n207 = local write "新密码"(w138) -> ()
            n208 = local write "旧密码"(w138) -> ()
          }
          event "用户管理": Mouse Up {
            n209 = event-data() -> ()  [unwired: 1 in, 1 out]
            n210 = call-poly <vilib>:"Delacor_lib_QMH_Enqueue Message (poly).vi"("Message"="in", "Message Queue in"=w150) -> ("error out"=w148:errorcluster, "Message Queue out"=w149:refnum<class "Delacor_lib_QMH_Message Queue.lvclass">)  [unwired: 8 in]
            n211 = call "Origin.vi"("error in"=w148, "数值 2"=0.0, "数值"=1750.0) -> ("error out"=w153:errorcluster)  [unwired: 8 in]
          }
          event "退出登录": Mouse Up {
            n212 = event-data() -> ()  [unwired: 1 in, 1 out]
            n213 = call "Stop Module.vi"("Wait for Module to Stop? (F)"=FALSE) -> ("error out"=w156:errorcluster)  [unwired: 10 in]
          }
          event "删除": Mouse Up {
            n214 = event-data() -> ()  [unwired: 1 in, 1 out]
            n215 = call-poly <vilib>:"Delacor_lib_QMH_Enqueue Message (poly).vi"("Message"="删除", "Message Queue in"=w162) -> ("error out"=w160:errorcluster, "Message Queue out"=w161:refnum<class "Delacor_lib_QMH_Message Queue.lvclass">)  [unwired: 8 in]
          }
          event "注册": Mouse Up {
            n216 = event-data() -> ()  [unwired: 1 in, 1 out]
            n217 = call "Origin.vi"("数值 2"=0.0, "数值"=2300.0) -> ("error out"=w164:errorcluster)  [unwired: 9 in]
          }
          event "管理返回": Mouse Up {
            n218 = event-data() -> ()  [unwired: 1 in, 1 out]
            n219 = call "Origin.vi"("数值 2"=0.0, "数值"=550.0) -> ("error out"=w171:errorcluster)  [unwired: 9 in]
          }
          event "注册确定": Mouse Up {
            n220 = event-data() -> ()  [unwired: 1 in, 1 out]
            n221 = call-poly <vilib>:"Delacor_lib_QMH_Enqueue Message (poly).vi"("Message"="注册确定", "Message Queue in"=w177) -> ("error out"=w175:errorcluster, "Message Queue out"=w176:refnum<class "Delacor_lib_QMH_Message Queue.lvclass">)  [unwired: 8 in]
          }
          event "注册取消": Mouse Up {
            n222 = event-data() -> ()  [unwired: 1 in, 1 out]
            n223 = call "Origin.vi"("数值 2"=0.0, "数值"=1750.0) -> ("error out"=w181:errorcluster)  [unwired: 9 in]
          }
          event "改密确定": Mouse Up {
            n224 = event-data() -> ()  [unwired: 1 in, 1 out]
            n225 = call-poly <vilib>:"Delacor_lib_QMH_Enqueue Message (poly).vi"("Message"="修改密码", "Message Queue in"=w187) -> ("error out"=w185:errorcluster, "Message Queue out"=w186:refnum<class "Delacor_lib_QMH_Message Queue.lvclass">)  [unwired: 8 in]
          }
          event "改密取消": Mouse Up {
            n226 = event-data() -> ()  [unwired: 1 in, 1 out]
            n227 = call "Origin.vi"("数值 2"=0.0, "数值"=550.0) -> ("error out"=w191:errorcluster)  [unwired: 9 in]
          }
          event "返回": Mouse Up {
            n228 = event-data() -> ()  [unwired: 1 in, 1 out]
            n229 = call-poly <vilib>:"Delacor_lib_QMH_Enqueue Message (poly).vi"("Message"="进入console", "Message Queue in"=w196) -> ("error out"=w195:errorcluster, "Message Queue out"=w197:refnum<class "Delacor_lib_QMH_Message Queue.lvclass">)  [unwired: 8 in]
          }
          event User Event {
            # "Another Module called the \"原点\" API Method."
            n230 = event-data() -> ("x"=w201:dbl, "y"=w200:dbl)  [unwired: 1 in]
            n231 = Bundle(cluster=T7 {"x"=0.0, "y"=0.0} ("原点 Argument"), "x"=w201, "y"=w200) -> (w202:T7)
            n232 = call-poly <vilib>:"Delacor_lib_QMH_Enqueue Message (poly).vi"("Message Data"=w202, "Message"="原点", "Message Queue in"=w207) -> ("error out"=w199:errorcluster, "Message Queue out"=w205:refnum<class "Delacor_lib_QMH_Message Queue.lvclass">)  [unwired: 7 in]
          }
          event User Event {
            # "Another Module called the \"hid_panl\" API Method."
            n233 = event-data() -> ("布尔"=w209:bool)  [unwired: 1 in]
            n234 = Bundle(cluster=T8 {"布尔"=FALSE} ("hid_panl Argument"), "布尔"=w209) -> (w210:T8)
            n235 = call-poly <vilib>:"Delacor_lib_QMH_Enqueue Message (poly).vi"("Message Data"=w210, "Message"="hid_panl", "Message Queue in"=w215) -> ("error out"=w208:errorcluster, "Message Queue out"=w213:refnum<class "Delacor_lib_QMH_Message Queue.lvclass">)  [unwired: 7 in]
          }
        }
        n236 = call-dynamic "Delacor_lib_QMH_Error Handler - Event Handling Loop.vi"("error in"=w54, "Message Queue in"=w52) -> ("dup error in"=w51:errorcluster)  [unwired: 8 in, 1 out]
      }
    }
    frame Error {
      # "Synchronize Caller Events.vi will inform Start Module.vi that the module has launched and will let the code calling Start Module.vi register for broadcasts and would permit the caller receive the broadcast that an error occurred at launch time."
      n237 = call "Synchronize Caller Events.vi"("Singleton Module Admin in"=w567) -> ("error out"=w564:errorcluster)  [unwired: 9 in, 1 out]
      n238 = call "Module Name--constant.vi"() -> ("Module Name"=w570:string)  [unwired: 11 in]
      n239 = Format Into String(format string="An error occurred during initialization. %s is no longer running.", w570) -> (resulting string=w568:string)  [unwired: 2 in, 1 out]
      n240 = Merge Errors(w566, w564) -> (w565:errorcluster)
      n241 = call "Error Reported.vi"("Additional Information"=w568, "Error"=w565) -> ()  [unwired: 9 in, 1 out]
    }
  }
  n242 = call "登录FGV.vi"("枚举"=enum16{"init", "quit", "read", "wirte"}."init") -> ("wirte 2"=w3:T13)  [unwired: 10 in]
  n243 = Unbundle By Name(w3) -> ("登录名"=w4:string)
  n244 = local write "密码"("" ("密码")) -> ()
  n245 = local write "用户名"(w4) -> ()
  n246 = Merge Errors(w10, w31) -> (w9:errorcluster)
  n247 = call "Close Module.vi"("error in (no error)"=w9, "Module Admin in"=w32) -> ("error out"=w25:errorcluster, "External Launch"=w22:bool, "Module Admin out"=w24:refnum<class "Delacor_lib_QMH_Module Admin.lvclass">)  [unwired: 7 in]
  n248 = Unregister For Events(event registration refnum=w30, error in=w25) -> (error out=w23:errorcluster)
  "error out" <- w23
  n249 = case "External Launch?" shown="真" w22 {
    tunnel: w23 -> [_ w576]
    tunnel: w20 -> [_ w575]
    tunnel: w15 -> [_ w573]
    frame False {
    }
    frame True {
      n250 = call-dynamic <vilib>:"Close.vi"("Panel In"=w575) -> ("Error Out"=w574:errorcluster)  [unwired: 10 in]
      n251 = call <vilib>:"Close.vi"("error in (no error)"=w574, "Controller in"=w573) -> ("error out"=w572:errorcluster)  [unwired: 9 in]
      n252 = case shown="错误" w576 {
        tunnel: w572 -> [_ _]
        frame No Error {
        }
        frame Error {
          n253 = invoke class="VI" method="FP.Open"("Activate"=TRUE ("Activate?")) -> ()  [unwired: 4 in, 5 out]
        }
      }
    }
  }
  n254 = local write "Module Admin"(w24) -> ()
